vi "Set MC Test Data Global.vi"(7 "Append Name":string, 8 "error in (no error)":errorcluster, 11 "Save MC TestData":bool) -> (0 "error out":errorcluster, 3 "Test GraphData Path":path)   [LabVIEW 2020]
uses:
  Global Variables/General Globals.vi
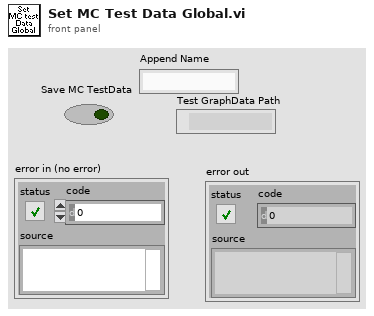
[diagram p1: front panel]
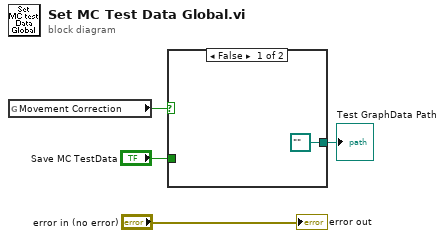
[diagram p0: block diagram]
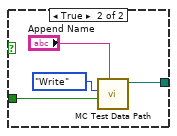
[diagram p2: hidden frame]
diagram:
  n1 = global read "General Globals.vi" "Movement Correction"() -> (w4:bool)
  n2 = case shown="False" w4 {
    tunnel: "Save MC TestData" -> [_ w8]
    tunnel: [path "" ("Test GraphData Path") w6] -> w1
    frame False {
    }
    frame True {
      n3 = call "MC Test Data Path.vi"("Append Name"="Append Name", "Save Test Data"=w8, "State"=enum16{"Initialise", "Write", "Read"}."Write") -> ("Test GraphData Path"=w6:path)  [unwired: 6 in, 2 out]
    }
  }
  "Test GraphData Path" <- w1
  "error out" <- "error in (no error)"
